vi "test--uniform_navy_000080_1x1.vi"(11 "Test Case In":refnum<class "PNG Determine Dominant Color.lvclass">) -> (0 "error out":errorcluster, 3 "Test Case Out":refnum<class "PNG Determine Dominant Color.lvclass">)   [LabVIEW 2021, in "PNG Determine Dominant Color.lvclass"]
uses:
  PNG Determine Dominant Color.lvclass
  C:/Program Files/National Instruments/LabVIEW 2026/vi.lib/Astemes/LUnit/Test Case.lvclass
  <vilib>/Astemes/LUnit/Test Case.lvclass/Test Case.ctl
  4993e8ee-a06a-463a-9684-69129f64d5ce.vi
  <vilib>/Astemes/LUnit/Core/LUnit Test Case/Private/Append Pass Result.vi
  <vilib>/Astemes/LUnit/Core/LUnit Test Case/Private/Append Fail Result.vi
  4993e8ee-a06a-463a-9684-69129f64d5ce.vi/9c5d11cd-9439-4240-a1ee-d9baace9c924.vi
  <vilib>/Astemes/LUnit/Core/LUnit Test Case/Private/Run In UI.vi
  <vilib>/Utility/error.llb/Clear Errors.vi
  src/Material SubVIs/Material SubVIs.lvlib
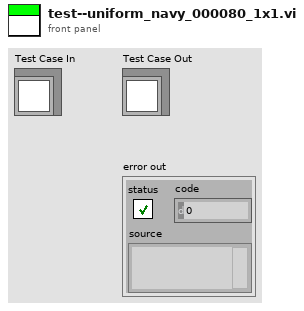
[diagram p1: front panel]
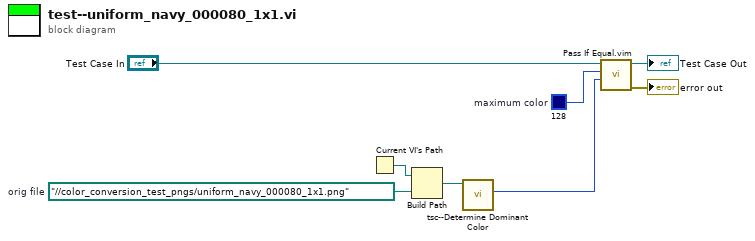
[diagram p0: block diagram]
diagram:
  w4 = u32 128  # maximum color
  w2 = path "../../color_conversion_test_pngs/uniform_navy_000080_1x1.png"  # orig file
  n1 = Current VI's Path() -> (path=w3:path)
  n2 = Build Path(base path=w3, name or relative path=w2) -> (appended path=w1:path)
  n3 = call "tsc--Determine Dominant Color.vi"("orig file"=w1) -> ("maximum color"=w5:u32)  [unwired: 8 in, 2 out]
  n4 = call "Pass If Equal.vim"("Actual"=w5, "Expected"=w4, "LUnit Test Case In"="Test Case In") -> ("error out"=→"error out":errorcluster, "LUnit Test Case Out"=→"Test Case Out":refnum<class "PNG Determine Dominant Color.lvclass">)  [unwired: 7 in]
